vi "get_chirp_point__e55fb91089.vi"(0 "relative seconds":dbl, 1 "omega2":dbl=1.0 format="%0.2f", 2 "Duration":dbl, 5 "voltage to displacement constant":dbl, 7 "Initial position in voltage":dbl, 9 "amplitude":dbl=1.0 format="%0.2f", 11 "omega1":dbl=1.0 format="%0.2f", 12 "r":dbl, 13 "waiting time (s)":dbl) -> (3 "set point":dbl, 14 "Elapsedf time (s)":dbl)   [LabVIEW 2023]
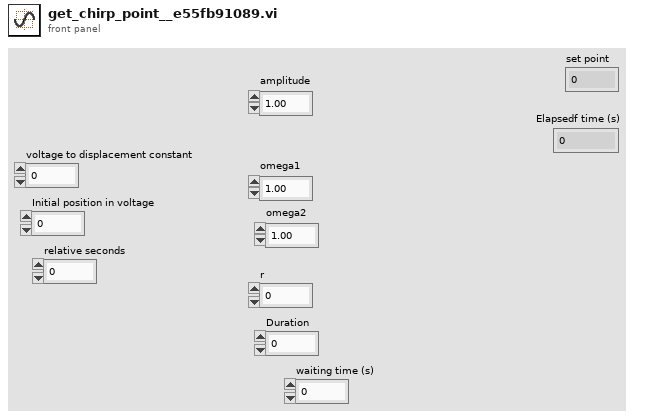
[diagram p1: front panel]
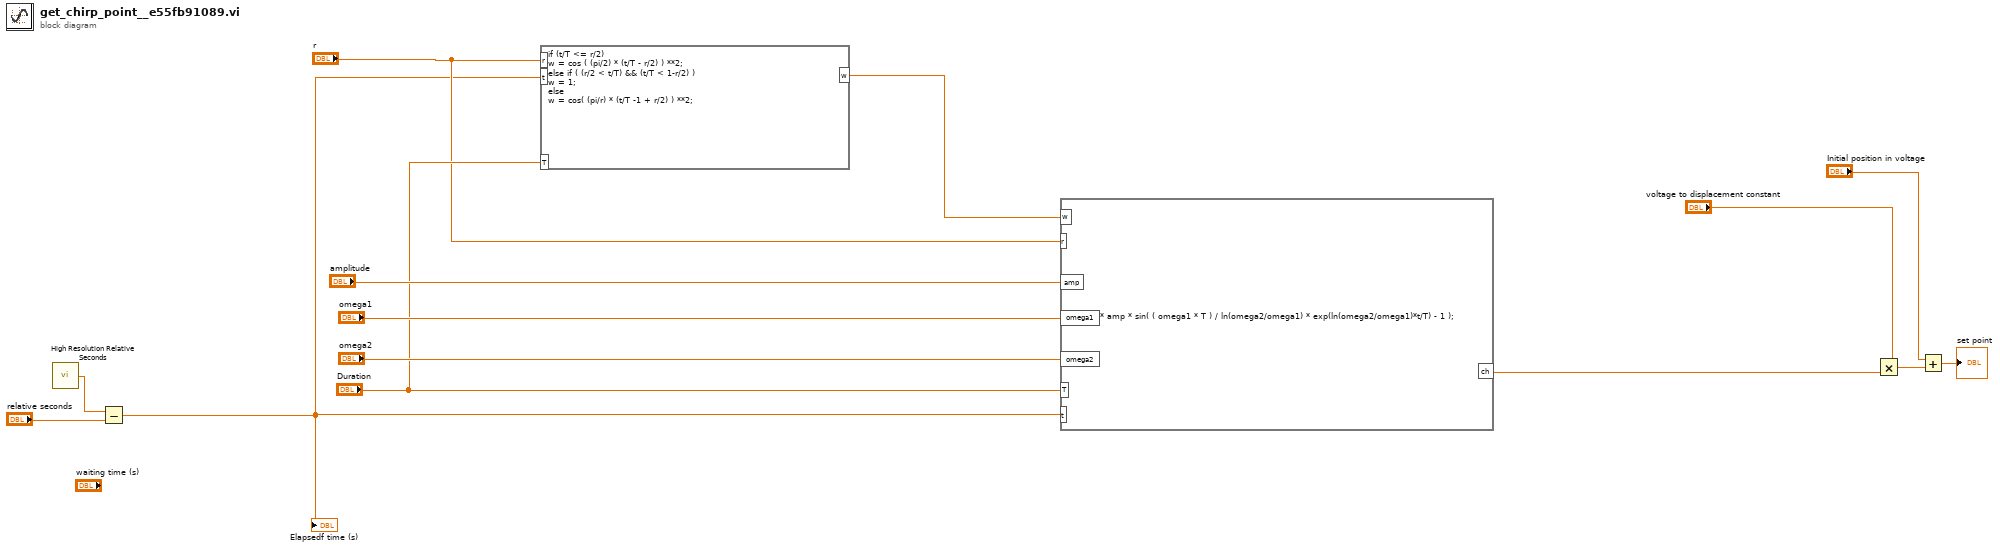
[diagram p0: block diagram]
diagram:
  n1 = call <vilib>:"High Resolution Relative Seconds.vi"() -> ("relative seconds"=w13:dbl)
  n2 = Subtract(x=w13, y="relative seconds") -> (x-y=w1:dbl)
  "Elapsedf time (s)" <- w1
  n3 = formula code="if (t/T <= r/2) \nw = cos ( (pi/2) * (t/T - r/2) ) **2;\nelse if ( (r/2 < t/T) && (t/T < 1-r/2) )\nw = 1;\nelse\nw = cos( (pi/r) * (t/T -1 + r/2) ) **2;"("r"="r", "t"=w1, "T"="Duration") -> ("w"=w2:dbl)
  n4 = formula code="ch = w * amp * sin( ( omega1 * T ) / ln(omega2/omega1) * exp(ln(omega2/omega1)*t/T) - 1 );"("amp"="amplitude", "omega1"="omega1", "omega2"="omega2", "T"="Duration", "t"=w1, "r"="r", "w"=w2) -> ("ch"=w8:dbl)
  n5 = Multiply(x="voltage to displacement constant", y=w8) -> (x*y=w10:dbl)
  n6 = Add(x="Initial position in voltage", y=w10) -> (x+y=→"set point":dbl)
